vi "Update Listbox Row.vi"(11 "cluster in":T1 {"DI"."Upper limit" format="%#_7f"; "DI"."Lower limit" format="%#_7f"}) -> (3 "cluster out":T1={"User name"="", "user account"="", "UI"=[], "DI"=[], "Barcode"="", "MCListbox Ref_in"=refnum, "sequence step #"=0, "Result?"=FALSE, "Report Path"=path "", "Test Sequence"=enum."Ensure all the connections are OK", "skip Test  "=[FALSE, FALSE, FALSE, FALSE, FALSE, FALSE, FALSE, FALSE, FALSE, FALSE, FALSE, FALSE, FALSE, FALSE, FALSE, FALSE, FALSE, FALSE, FALSE, FALSE, FALSE, FALSE, FALSE, FALSE, FALSE, FALSE, FALSE, FALSE, FALSE, FALSE, FALSE, FALSE]} {"DI"."Upper limit" format="%#_7f"; "DI"."Lower limit" format="%#_7f"})   [LabVIEW 2021]
uses:
  5.ACTIVITIES/1.LabVIEW_State_Machine_Template/LabVIEW_State_Machine_Template/LabVIEW_State_Machine_Template/Project_Template/Queue Test updator/Controls/initialise cluster.ctl
  5.ACTIVITIES/1.LabVIEW_State_Machine_Template/LabVIEW_State_Machine_Template/LabVIEW_State_Machine_Template/Project_Template/Queue Test updator/Controls/test step description.ctl
  5.ACTIVITIES/1.LabVIEW_State_Machine_Template/LabVIEW_State_Machine_Template/LabVIEW_State_Machine_Template/Project_Template/Queue Test updator/Controls/comparison selection.ctl
  controls/Main test sequence.ctl
  <vilib>/Utility/miscctls.llb/LVRowAndColumnUnsignedTypeDef.ctl
panel:
  out "sequence step #":u32
  out "updated row #":i32
  out "MCListbox Refnum out":refnum<vi>
  out "error out":errorcluster
  in  "error in":errorcluster
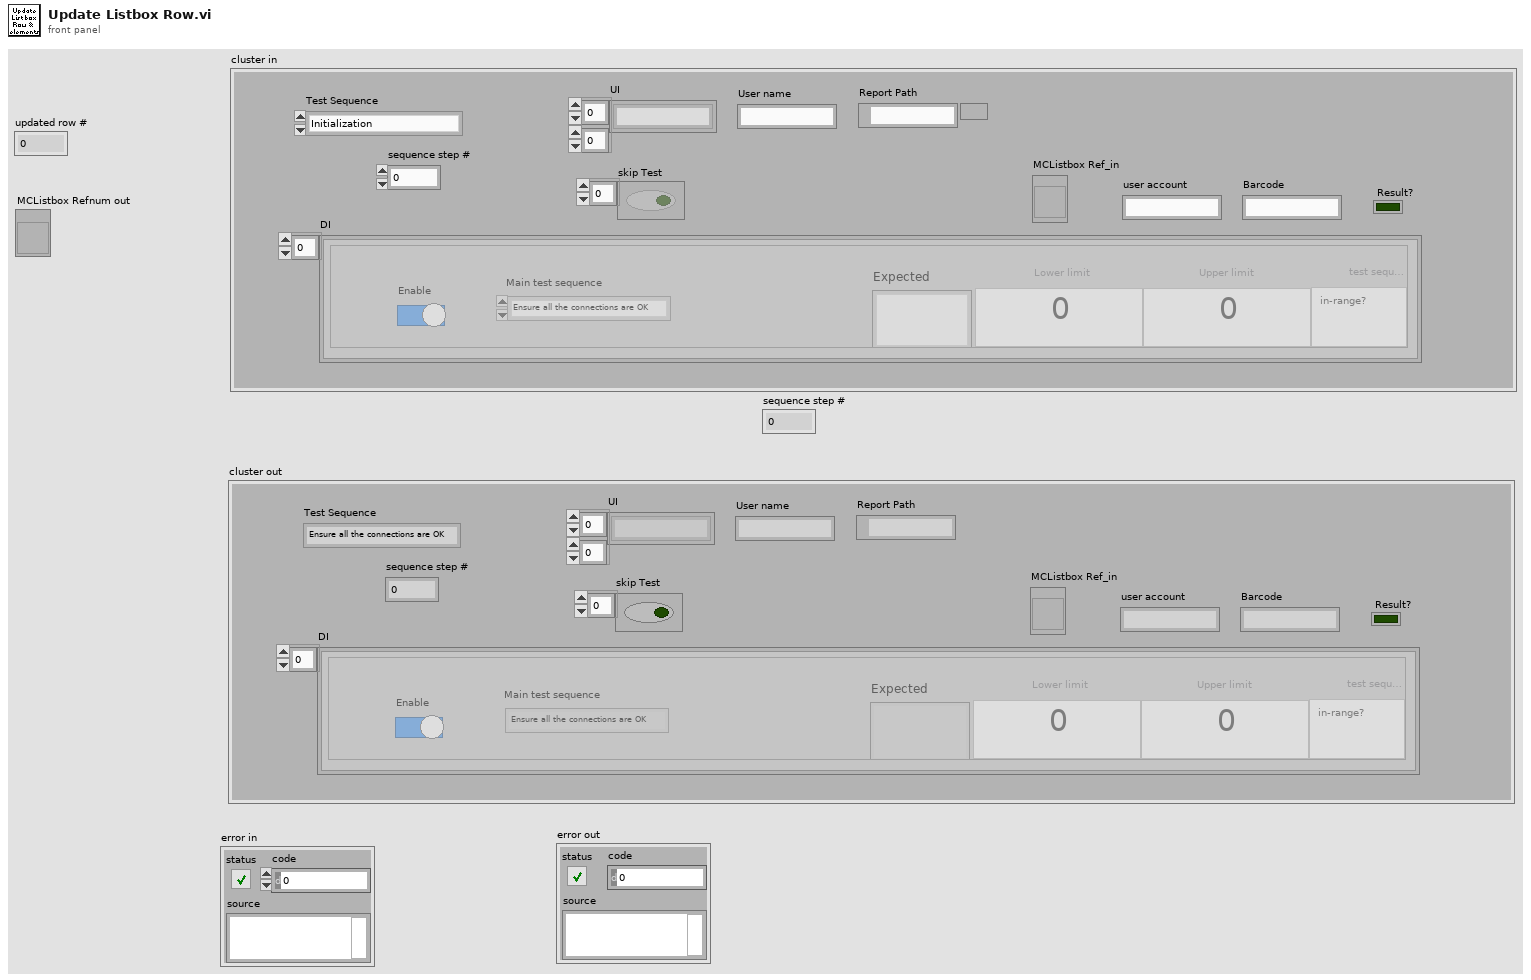
[diagram p1: front panel]
types:
  T1 = typedef "initialise cluster.ctl" = cluster{"User name":string, "user account":string, "UI":string[][], "DI":T2[], "Barcode":string, "MCListbox Ref_in":refnum<vi>, "sequence step #":u32, "Result?":bool, "Report Path":path, "Test Sequence":T4, "skip Test  ":bool[]}
  T2 = typedef "test step description.ctl" = cluster{"Lower limit":dbl, "Upper limit":dbl, "Comparison":T3, "Expected":string, "Enable":bool, "Main test sequence":T4}
  T3 = typedef "comparison selection.ctl" = enum16{"None", "in-range?", "less than?", "greater than?", "equal to?", "not equal to?", "less or equal to?", "greater or equal to?"}
  T4 = typedef "Main test sequence.ctl" = enum16{"Initialization", "Ensure all the connections are OK", "Turn ON 230V AC Input", "Load the Firmware", "Unlock_Opensesame & Stop console Logs", "Earth Detection", "Read Firmware", "Read & Write PCB Serial No", "Emergancy Switch Check", "Update WIFI credentials ", "Reboot", "Unlock Opensesame & Stop_console Logs", "WIFI State", "WIFI SSID", "Board revision", "ADC NTC Temp", "ADC_TYPE2_RCD_CURRENT", "5V Output Voltage", "3.3V Output Voltage", "D+M Sense", "Output Weld Sense", "FW Power Reset", "Unlock Opensesame & Stop console_Logs", "Reset switch Check", "Exit"}
  T5 = typedef "LVRowAndColumnUnsignedTypeDef.ctl" = cluster{"Row":u32, "Column":u32}
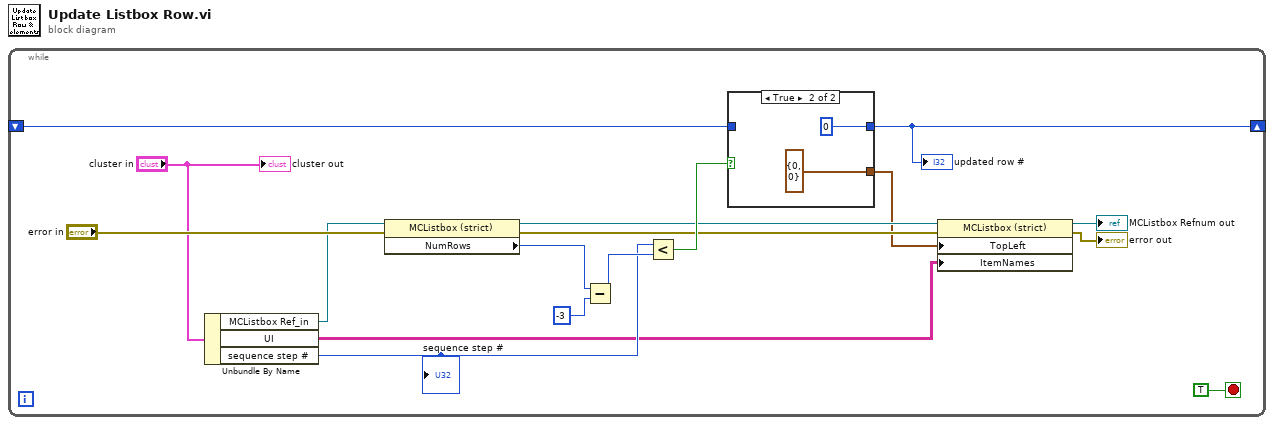
[diagram p0: block diagram]
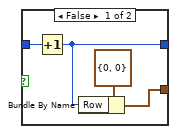
[diagram p2: hidden frame]
diagram:
  n1 = while {
    shift-right: [w7] -> _
    shift-left: _ -> [w8]
    stop <- TRUE stop-if-true
    n2 = Unbundle By Name("cluster in") -> ("MCListbox Ref_in"=w5:refnum<vi>, "UI"=w2:string[][], "sequence step #"=w3:u32)
    "sequence step #" <- w3
    n3 = property class="MCListbox (strict)"(reference=w5, error in="error in") -> (reference out=w11:refnum<vi>, error out=w10:errorcluster, "NumRows"=w6:u32)
    n4 = Subtract(x=w6, y=-3) -> (x-y=w13:u32)
    n5 = Less?(x=w3, y=w13) -> (x < y?=w12:bool)
    n6 = case shown="True" w12 {
      tunnel: [w20 T5 {"Row"=0, "Column"=0} ("Top Left Visible Cell")] -> w4
      tunnel: [w18 0] -> w7
      tunnel: w8 -> [w19 _]
      frame False {
        n7 = Increment(x=w19) -> (x+1=w18:i32)
        n8 = Bundle By Name(cluster=T5 {"Row"=0, "Column"=0} ("Top Left Visible Cell"), "Row"=w18) -> (w20:T5)
      }
      frame True {
      }
    }
    "updated row #" <- w7
    n9 = property class="MCListbox (strict)"(reference=w11, error in=w10, "TopLeft"=w4, "ItemNames"=w2) -> (reference out=→"MCListbox Refnum out":refnum<vi>, error out=→"error out":errorcluster)
    "cluster out" <- "cluster in"
  }
